vi "Main.vi"(11 "Module Admin":refnum<class "Delacor_lib_QMH_Module Admin.lvclass">) -> ()   [LabVIEW 2026, in "testCoordinator.lvlib"]
doc: "This template is based off of the Queued Message Handler design pattern and the Queued Message Handler project template that ships with LabVIEW.\n\nThe main difference is that the queue is private to this module and communication between modules is performed via Broadcast and Request events.\n\nRequest events are wrapped in public API methods and are handled in the Event Handling Loop (EHL) of this VI. Any module can register for Broadcast events sent by this module. The EHL generates messages based on user interface actions.\n\nThe Message Handling Loop (MHL) processes messages generated by the EHL, or by other messages. The messages are string values, so new messages can be added easily to the Message Cases case structure in the MHL. Each message cluster can also provide an optional value for Message Data, which is a variant that can be converted to whatever message-specific data is required.\n_____\nBased on DQMH Dev Tools: Project Template 7.1.2.1547."
uses:
  testCoordinator.lvlib
  <vilib>/Delacor/Delacor QMH/Libraries/Module Admin_class/Delacor_lib_QMH_Module Admin.lvclass
  Test Procedure.ctl
  modules/coordinator/src/Libraries/UserEventRecorder/TestEvent.ctl
  Module Data--cluster.ctl
  Do Something Argument--cluster.ctl
  <vilib>/Delacor/Delacor QMH/Libraries/Message Queue_class/Delacor_lib_QMH_Message Queue.lvclass/Delacor_lib_QMH_Message Queue.ctl
  Do Something Else Argument--cluster.ctl
  Do Something Else and Wait for Reply Argument--cluster.ctl
  Do Something Else and Wait (Reply Payload)--cluster.ctl
  Stop Argument--cluster.ctl
  <vilib>/Delacor/Delacor QMH/Libraries/Module Admin_class/Delacor_lib_QMH_Module Admin.lvclass/Delacor_lib_QMH_Module Admin.ctl
  Set Manual Tests Folder Location Argument--cluster.ctl
  Set Manual Tests Folder Location (Reply Payload)--cluster.ctl
  Load Test Procedure Argument--cluster.ctl
  Begin Test Execution Argument--cluster.ctl
  Process Test Procedure Metadata Argument--cluster.ctl
  Instruction Completed Argument--cluster.ctl
  Process First Instruction Argument--cluster.ctl
  Load Next Test Case Argument--cluster.ctl
  Execute Launcher Argument--cluster.ctl
  <vilib>/Utility/miscctls.llb/LVPointTypeDef.ctl
  modules/coordinator/src/Libraries/Launcher/Mode.ctl
  modules/ReplayMode.ctl
  modules/RecordMode.ctl
  <vilib>/Delacor/Delacor QMH/Libraries/Message Queue_class/Delacor_lib_QMH_Enqueue Message (Single).vi
  <vilib>/Delacor/Delacor QMH/Libraries/Module Admin_class/Delacor_lib_QMH_Get External Launch.vi
  modules/coordinator/src/Libraries/Core/global.vi
  <userlib>/_OpenG.lib/comparison/comparison.llb/String Changed__ogtk.vi
  <vilib>/Delacor/Delacor QMH/Libraries/Message Queue_class/Delacor_lib_QMH_Message Queue.lvclass
  modules/coordinator/src/Libraries/Launcher/Launcher.lvlib
  <userlib>/_OpenG.lib/comparison/comparison.llb/openg_comparison__ogtk.lvlib
panel:
  out "Array":T1[](array[typedef])
  in  "Exit":bool
  out "Scope":string
  out "TestProcedure":T2
  in  "Instruction Completed":bool
  out "Instruction":string
  out "Section":string
  out "Test Procedure":string
  out "error out":errorcluster
  out "X":dbl
  out "Status":string
  in  "Simulate MHL Error":bool
  in  "Simulate EHL Error":bool
  in  "Do Something Else <Replace Me>":bool
  in  "Do Something <Replace Me>":bool
  # "Open Visual Studio Code and run command \"LabVIEW Benchmark Actor: Capture LabVIEW Launch\" for the test to begin."
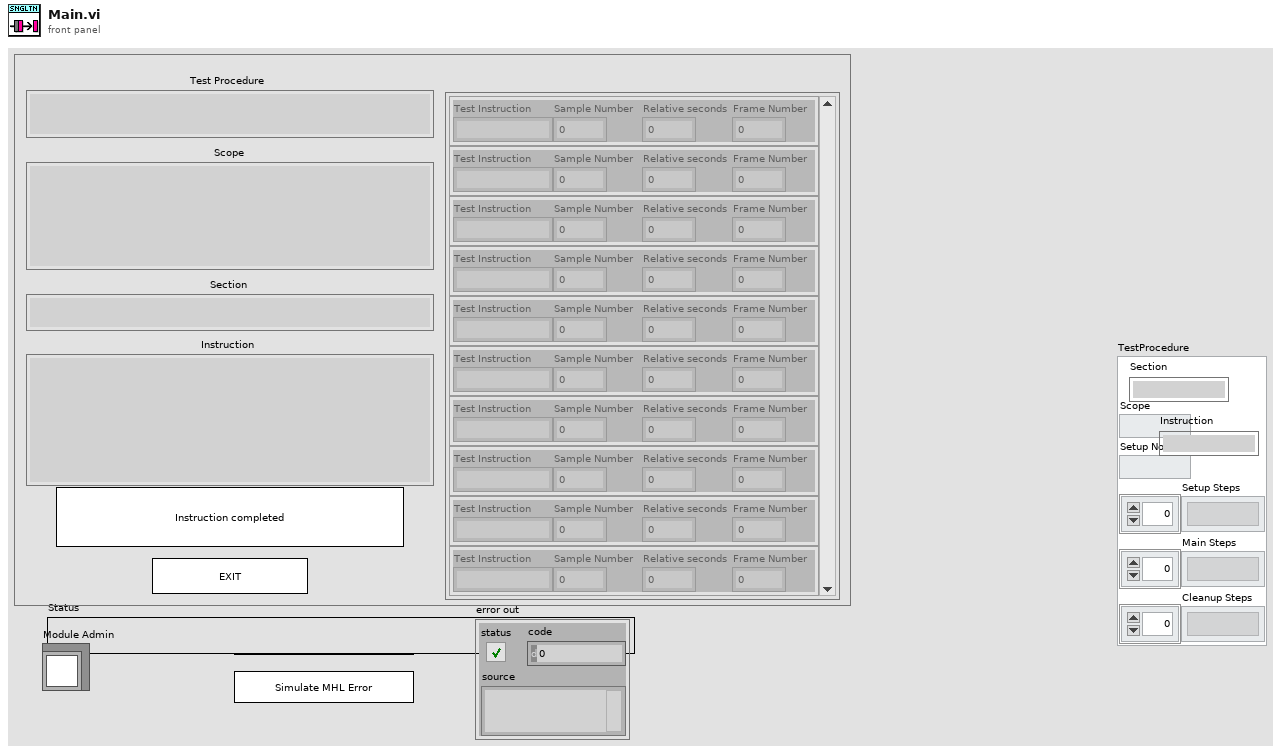
[diagram p1: front panel]
types:
  T1 = typedef "TestEvent.ctl" = cluster{"Test Instruction":string, "Sample Number":u32, "Relative seconds":dbl, "Frame Number":u32}
  T2 = typedef "Test Procedure.ctl" = cluster{"Scope":string, "Setup Note":string, "Setup Steps":string[], "Main Steps":string[], "Cleanup Steps":string[], "Section":string, "Instruction":string}
  T3 = typedef "testCoordinator.lvlib/Request Events--cluster.ctl" = cluster{"Stop Module":refnum<user-event>, "Do Something":refnum<user-event>, "Do Something Else":refnum<user-event>, "Do Something Else and Wait for Reply":refnum<user-event>, "Show Panel":refnum<user-event>, "Hide Panel":refnum<user-event>, "Get Module Execution Status":refnum<user-event>, "Show Diagram":refnum<user-event>, "Set Manual Tests Folder Location":refnum<user-event>, "Private.Load Test Procedure":refnum<user-event>, "Begin Test Execution":refnum<user-event>, "Private.Process Test Procedure Metadata":refnum<user-event>, "Private.Instruction Completed":refnum<user-event>, "Private.Process First Instruction":refnum<user-event>, "Private.Load Next Test Case":refnum<user-event>, "Private.Execute Launcher":refnum<user-event>}
  T4 = typedef "Launcher.lvlib/Broadcast Events--cluster.ctl" = cluster{"Module Did Init":refnum<user-event>, "Status Updated":refnum<user-event>, "Error Reported":refnum<user-event>, "Module Did Stop":refnum<user-event>, "Update Module Execution Status":refnum<user-event>, "Start Capture Detection Loop":refnum<user-event>, "Benchmark Started":refnum<user-event>, "Broadcast number of frames and run ID":refnum<user-event>}
  T5 = typedef "testCoordinator.lvlib/Module Data--cluster.ctl" = cluster{"Status":string, "Manual Tests Folder":path, "Available Tests":string[], "Test Procedure File Name":string, "TestCaseIndex":i32, "TestProcedure":T2}
  T6 = typedef "testCoordinator.lvlib/Do Something Argument--cluster.ctl" = cluster{"Do Something Msg":string}
  T7 = typedef "testCoordinator.lvlib/Do Something Else Argument--cluster.ctl" = cluster{"Do Something Else Msg":string, "X":dbl}
  T8 = typedef "testCoordinator.lvlib/Do Something Else and Wait for Reply Argument--cluster.ctl" = cluster{"Do Something Else Msg":string, "X":dbl, "Wait Notifier":refnum<notifier>, "wait for reply":bool}
  T9 = enum32{"invalid lock state", "Not Locked", "Locked (No Password)", "Password-protected"}
  T10 = typedef "testCoordinator.lvlib/Stop Argument--cluster.ctl" = cluster{"Origin":string, "Exit via Stop Module Req?":bool, "Wait for Module to stop?":bool}
  T11 = typedef "testCoordinator.lvlib/Set Manual Tests Folder Location Argument--cluster.ctl" = cluster{"Manual Tests Folder":path, "Wait Notifier":refnum<notifier>, "wait for reply":bool}
  T12 = typedef "testCoordinator.lvlib/Load Test Procedure Argument--cluster.ctl" = cluster{"Test Procedure File Name":string}
  T13 = typedef "testCoordinator.lvlib/Begin Test Execution Argument--cluster.ctl" = cluster{"Test Procedure":string}
  T14 = typedef "testCoordinator.lvlib/Process Test Procedure Metadata Argument--cluster.ctl" = cluster{"Boolean":bool}
  T15 = typedef "testCoordinator.lvlib/Instruction Completed Argument--cluster.ctl" = cluster{"Boolean":bool}
  T16 = typedef "testCoordinator.lvlib/Process First Instruction Argument--cluster.ctl" = cluster{"Boolean":bool}
  T17 = typedef "testCoordinator.lvlib/Load Next Test Case Argument--cluster.ctl" = cluster{"Boolean":bool}
  T18 = typedef "testCoordinator.lvlib/Execute Launcher Argument--cluster.ctl" = cluster{"Boolean":bool}
  T19 = typedef "LVPointTypeDef.ctl" = cluster{"Horizontal":i16, "Vertical":i16}
  T20 = enum32{"Invalid", "Standard", "Closed", "Hidden", "Minimized", "Maximized"}
  T21 = typedef "testCoordinator.lvlib/Do Something Else and Wait (Reply Payload)--cluster.ctl" = cluster{"Value":dbl, "error":errorcluster}
  T22 = typedef "testCoordinator.lvlib/Set Manual Tests Folder Location (Reply Payload)--cluster.ctl" = cluster{"Available Test Procedures":string[], "error":errorcluster}
  T23 = typedef "Mode.ctl" = cluster{"Replay":T24, "Record":T25}
  T24 = typedef "ReplayMode.ctl" = enum16{"None", "User Events"}
  T25 = typedef "RecordMode.ctl" = enum16{"None", "User Events", "Benchmarks", "User Events and Benchmarks"}
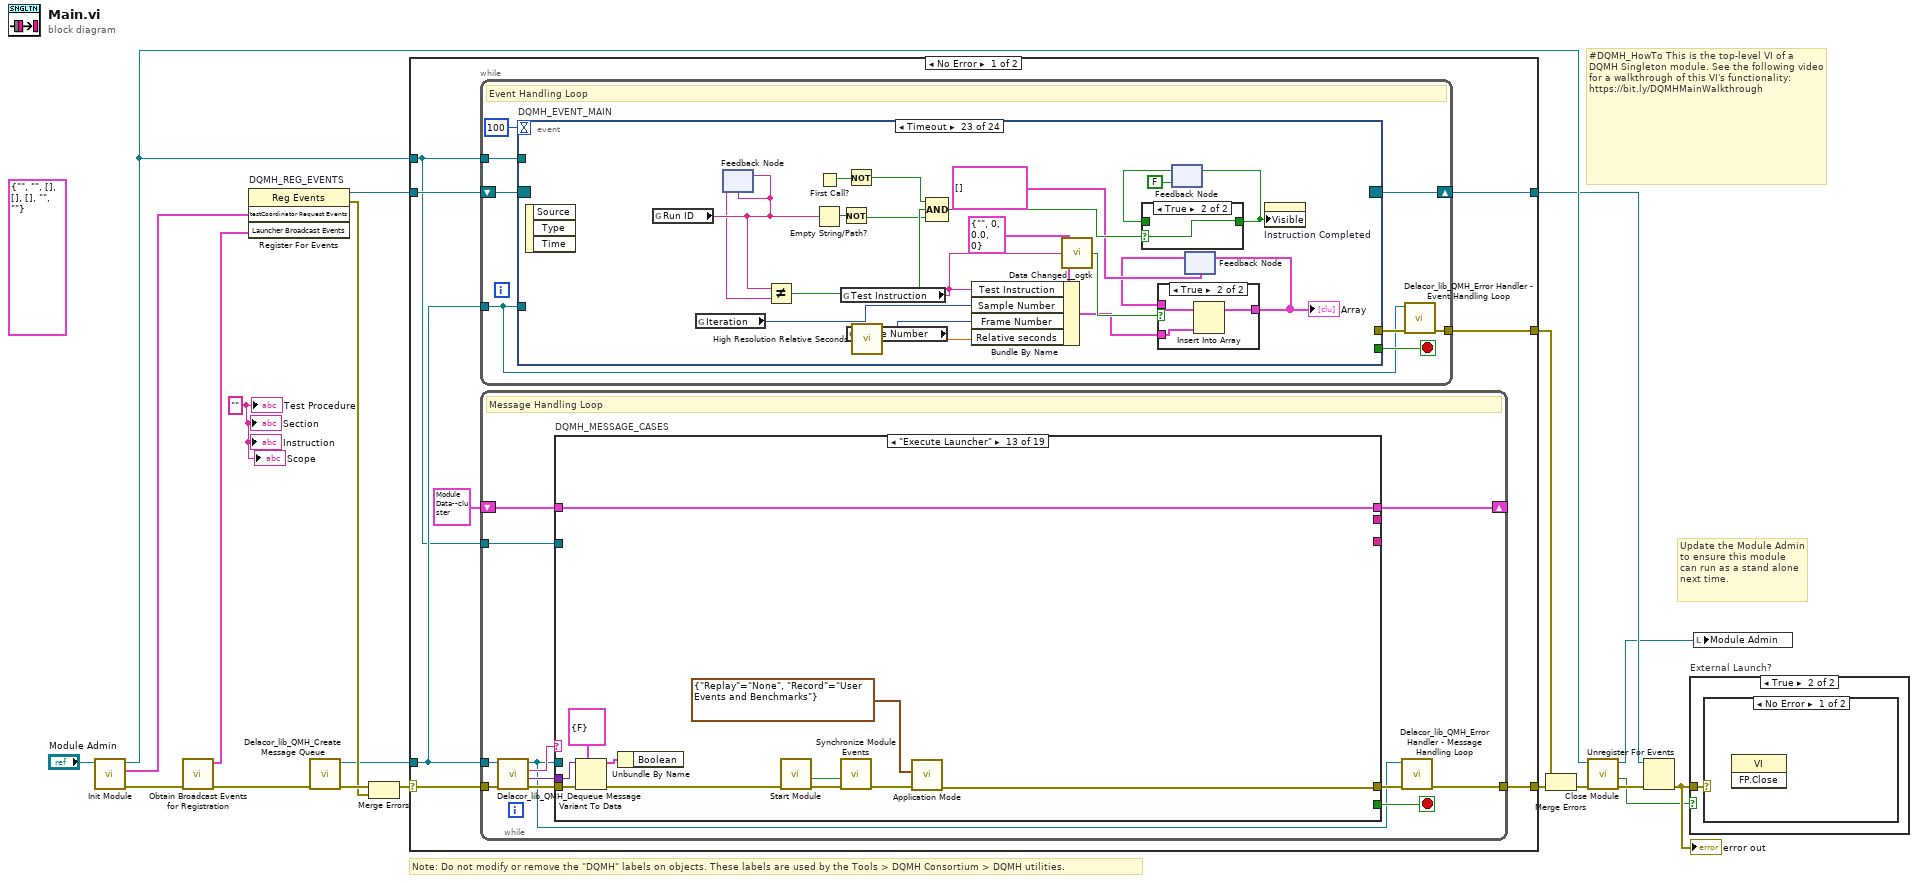
[diagram p0: block diagram]
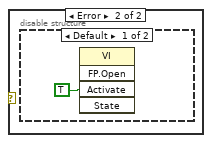
[diagram p3: hidden frame]
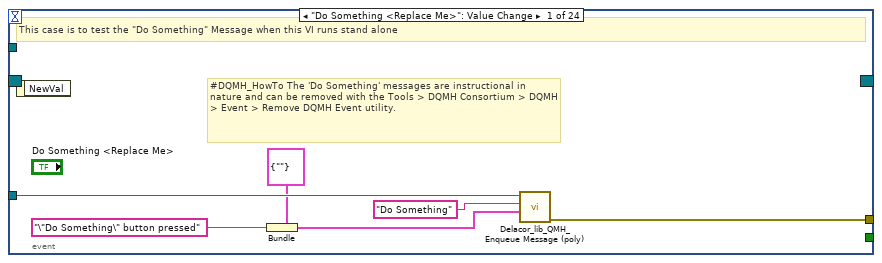
[diagram p5: hidden frame]
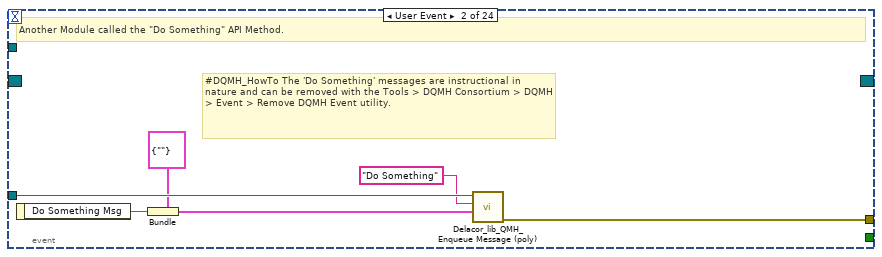
[diagram p6: hidden frame]
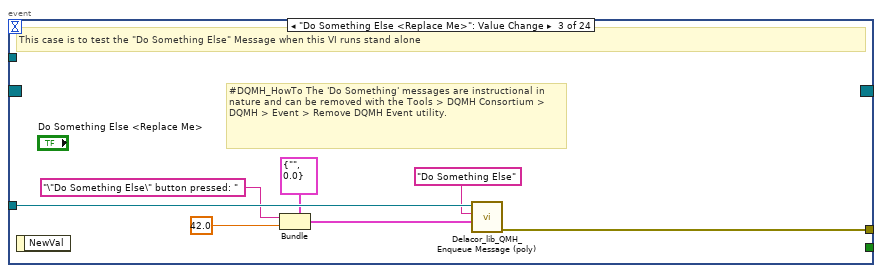
[diagram p7: hidden frame]
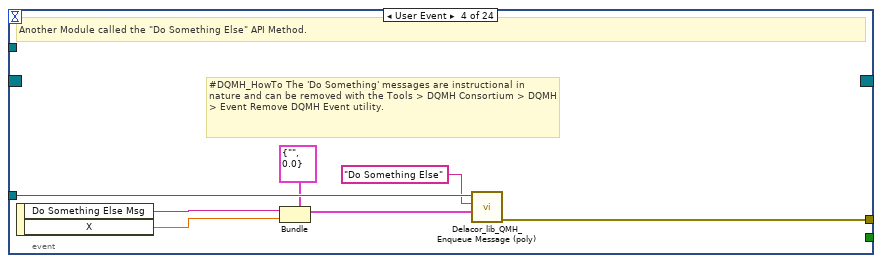
[diagram p8: hidden frame]
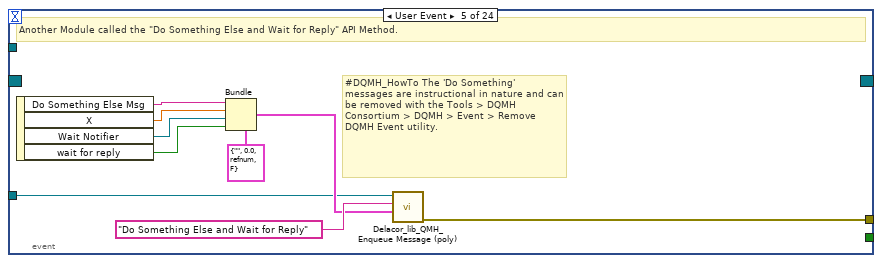
[diagram p9: hidden frame]
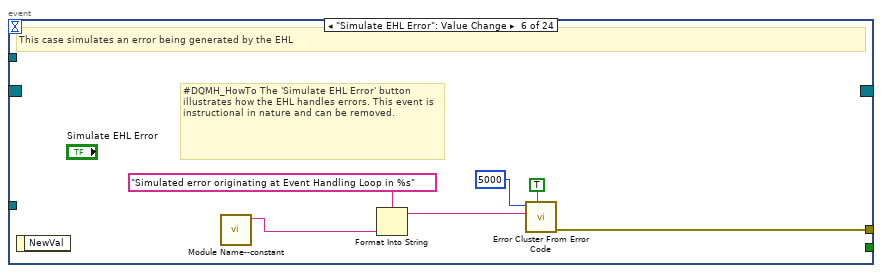
[diagram p10: hidden frame]
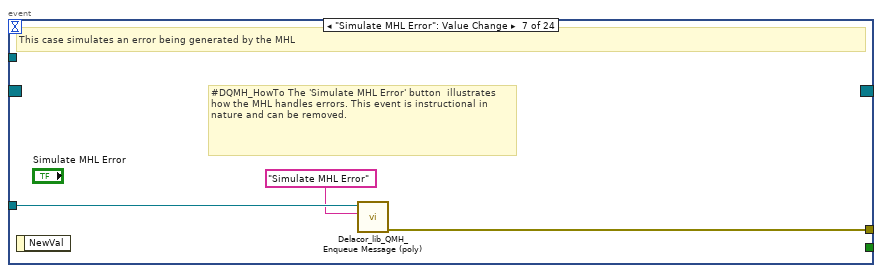
[diagram p11: hidden frame]
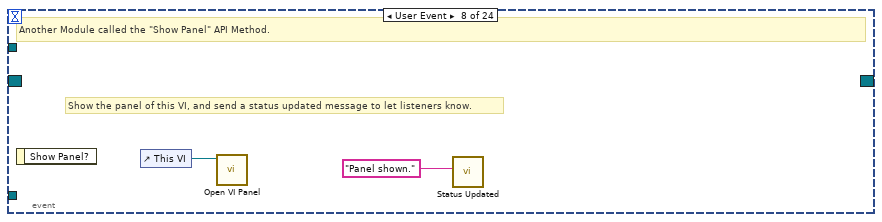
[diagram p12: hidden frame]
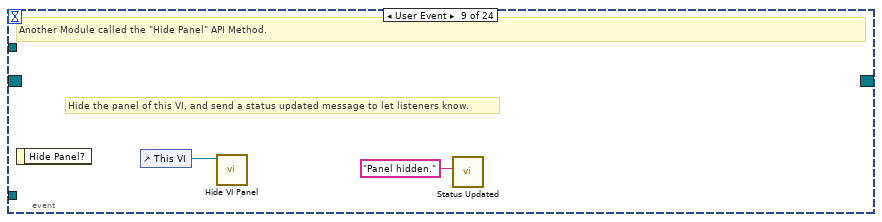
[diagram p13: hidden frame]
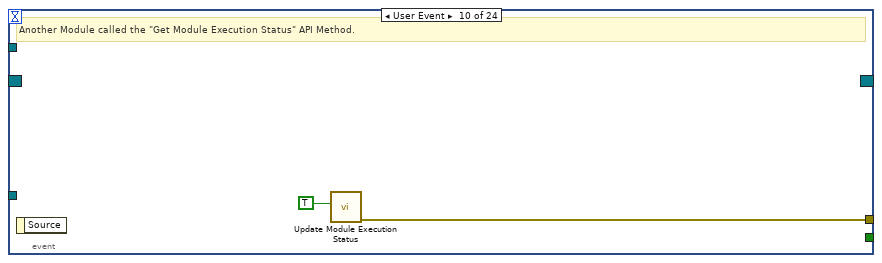
[diagram p14: hidden frame]
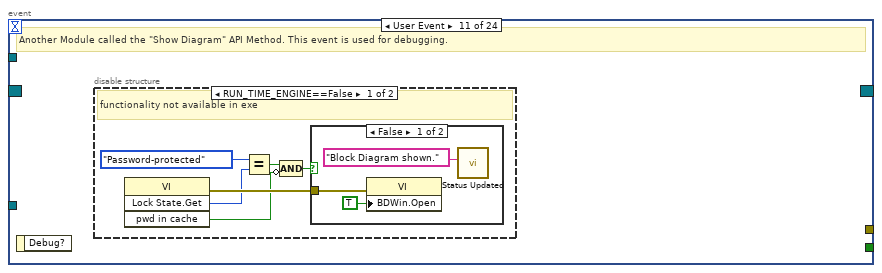
[diagram p15: hidden frame]
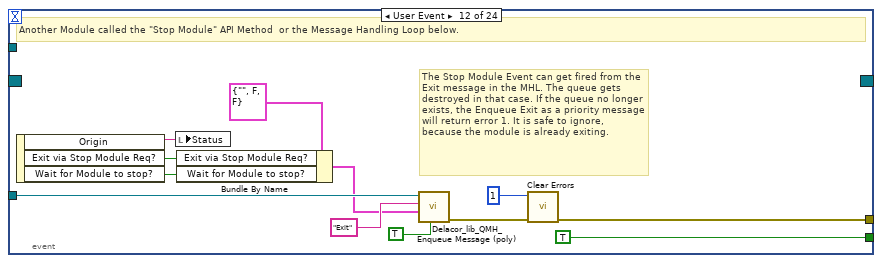
[diagram p18: hidden frame]
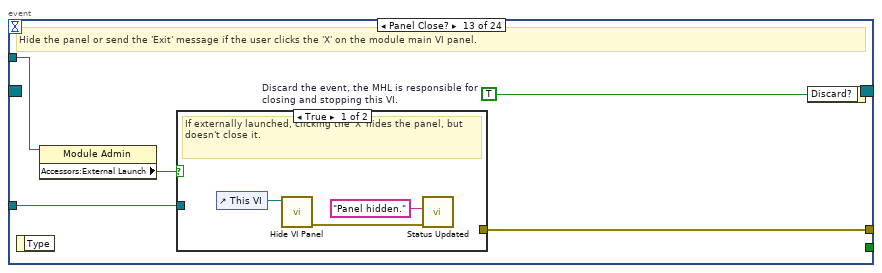
[diagram p19: hidden frame]
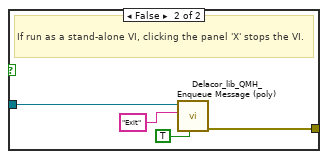
[diagram p20: hidden frame]
diagram:
  (unwired) T2 {"Scope"="", "Setup Note"="", "Setup Steps"=[], "Main Steps"=[], "Cleanup Steps"=[], "Section"="", "Instruction"=""} ("TestProcedure")
  w1 = "" ("Test Procedure")
  # "#DQMH_HowTo This is the top-level VI of a DQMH Singleton module. See the following video for a walkthrough of this VI's functionality: https://bit.ly/DQMHMainWalkthrough"
  # "Note: Do not modify or remove the \"DQMH\" labels on objects. These labels are used by the Tools > DQMH Consortium > DQMH utilities."
  # "Update the Module Admin to ensure this module can run as a stand alone next time."
  n1 = call "Init Module.vi"("Singleton Module Admin in"="Module Admin") -> ("error out"=w4:errorcluster, "testCoordinator Request Events"=w9:T3, "Singleton Module Admin out"=w12:refnum<class "Delacor_lib_QMH_Module Admin.lvclass">)  [unwired: 8 in]
  n2 = call "Obtain Broadcast Events for Registration.vi"("error in"=w4) -> ("error out"=w3:errorcluster, "Launcher Broadcast Events"=w2:T4)  [unwired: 8 in, 1 out]
  n3 = register-events "DQMH_REG_EVENTS"(w9, w2) -> (reference out=w10:refnum<event-registration>, error out=w13:errorcluster)  [unwired: 2 in]
  n4 = call <vilib>:"Delacor_lib_QMH_Create Message Queue.vi"("error in"=w3) -> ("error out"=w15:errorcluster, "Message Queue"=w8:refnum<class "Delacor_lib_QMH_Message Queue.lvclass">)  [unwired: 9 in]
  n5 = Merge Errors(w15, w13) -> (w14:errorcluster)
  n6 = case shown="No Error" w14 {
    selector: w14 -> [w26 w455]
    tunnel: [w28 w454] -> w20
    tunnel: [w25 w453] -> w11
    tunnel: w10 -> [w23 w453]
    tunnel: w8 -> [w22 w448]
    tunnel: [w27 _] -> w18
    tunnel: w12 -> [w21 w449]
    frame No Error {
      n7 = while {
        tunnel: w22 -> [w30]
        shift-right: [w33] -> w25
        shift-left: w23 -> [w34]
        tunnel: [w35] -> w27
        tunnel: w21 -> [w31]
        stop <- w32 stop-if-true
        # "Event Handling Loop"
        n8 = event "DQMH_EVENT_MAIN" shown="[22] Timeout" {
          selector: w34 -> [_ _ _ _ _ _ _ _ _ _ _ _ _ _ _ _ _ _ _ _ _ _ _ _]
          dyn-events: [_ _ _ _ _ _ _ _ _ _ _ _ _ _ _ _ _ _ _ _ _ _ _ _] -> w33
          timeout: 100 -> [_ _ _ _ _ _ _ _ _ _ _ _ _ _ _ _ _ _ _ _ _ _ _ _]
          tunnel: [_ _ _ _ _ _ _ _ _ _ _ TRUE ("Discard?") _ _ _ _ _ _ _ _ _ _ _ _] -> w32
          tunnel: w30 -> [w41 w47 w54 w61 w64 _ w79 _ _ _ _ w103 w110 w127 w133 w139 w145 w151 _ w158 w164 w170 _ _]
          tunnel: [w42 w48 w55 w62 w71 w77 w80 _ _ w86 _ w106 w112 w120 w128 w134 w140 w146 w152 w153 w159 w165 _ w198] -> w36
          tunnel: w31 -> [_ _ _ _ _ _ _ _ _ _ _ _ w109 _ _ _ _ _ _ _ _ _ _ _]
          event "Do Something <Replace Me>": Value Change {
            # "#DQMH_HowTo The 'Do Something' messages are instructional in nature and can be removed with the Tools > DQMH Consortium > DQMH > Event > Remove DQMH Event utility."
            # "This case is to test the \"Do Something\" Message when this VI runs stand alone"
            n9 = event-data() -> ()  [unwired: 1 in, 1 out]
            n10 = Bundle(cluster=T6 {"Do Something Msg"=""} ("Do Something Argument"), "Do Something Msg"="\"Do Something\" button pressed" ("\"Do Something\" button pressed")) -> (w37:T6)
            n11 = call-poly <vilib>:"Delacor_lib_QMH_Enqueue Message (poly).vi"("Message Data"=w37, "Message"="Do Something", "Message Queue in"=w41) -> ("error out"=w42:errorcluster)  [unwired: 7 in, 1 out]
          }
          event User Event {
            # "#DQMH_HowTo The 'Do Something' messages are instructional in nature and can be removed with the Tools > DQMH Consortium > DQMH > Event > Remove DQMH Event utility."
            # "Another Module called the \"Do Something\" API Method."
            n12 = event-data() -> ("Do Something Msg"=w44:string)  [unwired: 1 in]
            n13 = Bundle(cluster=T6 {"Do Something Msg"=""} ("Do Something Argument"), "Do Something Msg"=w44) -> (w43:T6)
            n14 = call-poly <vilib>:"Delacor_lib_QMH_Enqueue Message (poly).vi"("Message Data"=w43, "Message"="Do Something", "Message Queue in"=w47) -> ("error out"=w48:errorcluster)  [unwired: 7 in, 1 out]
          }
          event "Do Something Else <Replace Me>": Value Change {
            # "#DQMH_HowTo The 'Do Something' messages are instructional in nature and can be removed with the Tools > DQMH Consortium > DQMH > Event > Remove DQMH Event utility."
            # "This case is to test the \"Do Something Else\" Message when this VI runs stand alone"
            n15 = event-data() -> ()  [unwired: 1 in, 1 out]
            n16 = Bundle(cluster=T7 {"Do Something Else Msg"="", "X"=0.0} ("Do Something Else Argument"), "Do Something Else Msg"="\"Do Something Else\" button pressed: " ("\"Do Something Else\" button pressed"), "X"=42.0) -> (w51:T7)
            n17 = call-poly <vilib>:"Delacor_lib_QMH_Enqueue Message (poly).vi"("Message Data"=w51, "Message"="Do Something Else", "Message Queue in"=w54) -> ("error out"=w55:errorcluster)  [unwired: 7 in, 1 out]
          }
          event User Event {
            # "#DQMH_HowTo The 'Do Something' messages are instructional in nature and can be removed with the Tools > DQMH Consortium > DQMH > Event Remove DQMH Event utility."
            # "Another Module called the \"Do Something Else\" API Method."
            n18 = event-data() -> ("Do Something Else Msg"=w57:string, "X"=w56:dbl)  [unwired: 1 in]
            n19 = Bundle(cluster=T7 {"Do Something Else Msg"="", "X"=0.0} ("Do Something Else Argument"), "Do Something Else Msg"=w57, "X"=w56) -> (w58:T7)
            n20 = call-poly <vilib>:"Delacor_lib_QMH_Enqueue Message (poly).vi"("Message Data"=w58, "Message"="Do Something Else", "Message Queue in"=w61) -> ("error out"=w62:errorcluster)  [unwired: 7 in, 1 out]
          }
          event User Event {
            # "#DQMH_HowTo The 'Do Something' messages are instructional in nature and can be removed with the Tools > DQMH Consortium > DQMH > Event > Remove DQMH Event utility."
            # "Another Module called the \"Do Something Else and Wait for Reply\" API Method."
            n21 = event-data() -> ("Do Something Else Msg"=w67:string, "X"=w66:dbl, "Wait Notifier"=w65:refnum<notifier>, "wait for reply"=w63:bool)  [unwired: 1 in]
            n22 = Bundle(cluster=T8 {"Do Something Else Msg"="", "X"=0.0, "Wait Notifier"=refnum, "wait for reply"=FALSE} ("Do Something Else and Wait for Reply Argument"), "Do Something Else Msg"=w67, "X"=w66, "Wait Notifier"=w65, "wait for reply"=w63) -> (w68:T8)
            n23 = call-poly <vilib>:"Delacor_lib_QMH_Enqueue Message (poly).vi"("Message Data"=w68, "Message"="Do Something Else and Wait for Reply", "Message Queue in"=w64) -> ("error out"=w71:errorcluster)  [unwired: 7 in, 1 out]
          }
          event "Simulate EHL Error": Value Change {
            # "#DQMH_HowTo The 'Simulate EHL Error' button  illustrates how the EHL handles errors. This event is instructional in nature and can be removed."
            # "This case simulates an error being generated by the EHL"
            n24 = event-data() -> ()  [unwired: 1 in, 1 out]
            n25 = call "Module Name--constant.vi"() -> ("Module Name"=w74:string)  [unwired: 11 in]
            n26 = Format Into String(format string="Simulated error originating at Event Handling Loop in %s", w74) -> (resulting string=w75:string)  [unwired: 2 in, 1 out]
            n27 = call <vilib>:"Error Cluster From Error Code.vi"("show call chain? (False)"=TRUE, "error message (\"\")"=w75, "error code (0)"=5000) -> ("error out"=w77:errorcluster)  [unwired: 6 in]
          }
          event "Simulate MHL Error": Value Change {
            # "#DQMH_HowTo The 'Simulate MHL Error' button  illustrates how the MHL handles errors. This event is instructional in nature and can be removed."
            # "This case simulates an error being generated by the MHL"
            n28 = event-data() -> ()  [unwired: 1 in, 1 out]
            n29 = call-poly <vilib>:"Delacor_lib_QMH_Enqueue Message (poly).vi"("Message"="Simulate MHL Error", "Message Queue in"=w79) -> ("error out"=w80:errorcluster)  [unwired: 8 in, 1 out]
          }
          event User Event {
            # "Show the panel of this VI, and send a status updated message to let listeners know."
            # "Another Module called the \"Show Panel\" API Method."
            n30 = event-data() -> ()  [unwired: 1 in, 1 out]
            n31 = control-ref of="This VI"() -> (w82:refnum<vi>)
            n32 = call "Open VI Panel.vi"("VI"=w82) -> ()  [unwired: 10 in, 1 out]
            n33 = call "Status Updated.vi"("Status"="Panel shown." ("format string")) -> ()  [unwired: 10 in, 1 out]
          }
          event User Event {
            # "Hide the panel of this VI, and send a status updated message to let listeners know."
            # "Another Module called the \"Hide Panel\" API Method."
            n34 = event-data() -> ()  [unwired: 1 in, 1 out]
            n35 = control-ref of="This VI"() -> (w84:refnum<vi>)
            n36 = call "Hide VI Panel.vi"("VI"=w84) -> ()  [unwired: 10 in, 1 out]
            n37 = call "Status Updated.vi"("Status"="Panel hidden." ("format string")) -> ()  [unwired: 10 in, 1 out]
          }
          event User Event {
            # "Another Module called the \"Get Module Execution Status\" API Method."
            n38 = event-data() -> ()  [unwired: 1 in, 1 out]
            n39 = call "Update Module Execution Status.vi"("Running?"=TRUE) -> ("error out"=w86:errorcluster)  [unwired: 10 in]
          }
          event User Event {
            # "Another Module called the \"Show Diagram\" API Method. This event is used for debugging."
            n40 = event-data() -> ()  [unwired: 1 in, 1 out]
            n41 = disable-structure shown="RUN_TIME_ENGINE==False" {
              frame condition #0 (active) {
                # "functionality not available in exe"
                n42 = invoke on="Invoke Node" class="VI" method="Lock State.Get"() -> (error out=w92:errorcluster, "Get Lock State"=w91:T9, "pwd in cache"=w88:bool)  [unwired: 4 in, 1 out]
                n43 = Equal?(x=T9."Password-protected", y=w91) -> (x = y?=w89:bool)
                n44 = Compound Arithmetic op=AND(w89, invert w88) -> (w87:bool)
                n45 = case shown="False" w87 {
                  tunnel: w92 -> [w95 _]
                  frame False {
                    n46 = property on="Property Node" class="VI"(error in=w95, "BDWin.Open"=TRUE ("Block Diagram Window:Open")) -> ()  [unwired: 1 in, 2 out]
                    n47 = call "Status Updated.vi"("Status"="Block Diagram shown." ("format string")) -> ()  [unwired: 10 in, 1 out]
                  }
                  frame True {
                    # "Password-protected VI, and the password is not in the cache. Do not show the diagram."
                  }
                }
              }
              frame condition #1 {
              }
            }
          }
          event User Event {
            # "The Stop Module Event can get fired from the Exit message in the MHL. The queue gets destroyed in that case. If the queue no longer exists, the Enqueue Exit as a priority message will return error 1. It is safe to ignore, because the module is already exiting."
            # "Another Module called the \"Stop Module\" API Method  or the Message Handling Loop below."
            n48 = event-data() -> ("Origin"=w102:string, "Exit via Stop Module Req?"=w98:bool, "Wait for Module to stop?"=w97:bool)  [unwired: 1 in]
            n49 = local write "Status"(w102) -> ()
            n50 = Bundle By Name(cluster=T10 {"Origin"="", "Exit via Stop Module Req?"=FALSE, "Wait for Module to stop?"=FALSE} ("Stop Argument"), "Exit via Stop Module Req?"=w98, "Wait for Module to stop?"=w97) -> (w96:T10)
            n51 = call-poly <vilib>:"Delacor_lib_QMH_Enqueue Message (poly).vi"("Priority Message? (F)"=TRUE, "Message Data"=w96, "Message"="Exit", "Message Queue in"=w103) -> ("error out"=w107:errorcluster)  [unwired: 6 in, 1 out]
            n52 = call <vilib>:"Clear Errors.vi"("error in (no error)"=w107, "specific error code to clear (0: all)"=1) -> ("error out"=w106:errorcluster)  [unwired: 4 in, 1 out]
          }
          event Panel Close? {
            w111 = TRUE  # Discard the event, the MHL is responsible for closing and stopping this VI.
            # "Hide the panel or send the 'Exit' message if the user clicks the 'X' on the module main VI panel."
            n53 = event-data() -> ()  [unwired: 1 in, 1 out]
            n54 = property on="Property Node" class="Module Admin"(reference=w109) -> ("Accessors:External Launch"=w108:bool)  [unwired: 1 in, 2 out]
            n55 = case shown="True" w108 {
              tunnel: w110 -> [_ w118]
              tunnel: [_ w119] -> w112
              frame True {
                # "If externally launched, clicking the 'X' hides the panel, but doesn't close it."
                n56 = control-ref of="This VI"() -> (w115:refnum<vi>)
                n57 = call "Hide VI Panel.vi"("VI"=w115) -> ("error out"=w113:errorcluster)  [unwired: 10 in]
                n58 = call "Status Updated.vi"("error in"=w113, "Status"="Panel hidden." ("format string")) -> ()  [unwired: 9 in, 1 out]
              }
              frame False {
                # "If run as a stand-alone VI, clicking the panel 'X' stops the VI."
                n59 = call-poly <vilib>:"Delacor_lib_QMH_Enqueue Message (poly).vi"("Priority Message? (F)"=TRUE, "Message"="Exit", "Message Queue in"=w118) -> ("error out"=w119:errorcluster)  [unwired: 7 in, 1 out]
              }
            }
            n60 = event-data ("Event Filter Node")("Discard?"=w111) -> ()  [unwired: 1 in, 1 out]
          }
          event User Event {
            # "Another Module called the \"Set Manual Tests Folder Location\" API Method."
            n61 = event-data() -> ("Manual Tests Folder"=w123:path, "Wait Notifier"=w122:refnum<notifier>, "wait for reply"=w121:bool)  [unwired: 1 in]
            n62 = Bundle(cluster=T11 {"Manual Tests Folder"=path "", "Wait Notifier"=refnum, "wait for reply"=FALSE} ("Set Manual Tests Folder Location Argument"), "Manual Tests Folder"=w123, "Wait Notifier"=w122, "wait for reply"=w121) -> (w124:T11)
            n63 = call-poly <vilib>:"Delacor_lib_QMH_Enqueue Message (poly).vi"("Message Data"=w124, "Message"="Set Manual Tests Folder Location", "Message Queue in"=w127) -> ("error out"=w120:errorcluster)  [unwired: 7 in, 1 out]
          }
          event User Event {
            # "This module called the \"Private.Load Test Procedure\" private request."
            n64 = event-data() -> ("Test Procedure File Name"=w129:string)  [unwired: 1 in]
            n65 = Bundle(cluster=T12 {"Test Procedure File Name"=""} ("Load Test Procedure Argument"), "Test Procedure File Name"=w129) -> (w130:T12)
            n66 = call-poly <vilib>:"Delacor_lib_QMH_Enqueue Message (poly).vi"("Message Data"=w130, "Message"="Load Test Procedure", "Message Queue in"=w133) -> ("error out"=w128:errorcluster)  [unwired: 7 in, 1 out]
          }
          event User Event {
            # "Another Module called the \"Begin Test Execution\" API Method."
            n67 = event-data() -> ("Test Procedure"=w135:string)  [unwired: 1 in]
            n68 = Bundle(cluster=T13 {"Test Procedure"=""} ("Begin Test Execution Argument"), "Test Procedure"=w135) -> (w136:T13)
            n69 = call-poly <vilib>:"Delacor_lib_QMH_Enqueue Message (poly).vi"("Message Data"=w136, "Message"="Begin Test Execution", "Message Queue in"=w139) -> ("error out"=w134:errorcluster)  [unwired: 7 in, 1 out]
          }
          event User Event {
            # "This module called the \"Private.Process Test Procedure Metadata\" private request."
            n70 = event-data() -> ("Boolean"=w141:bool)  [unwired: 1 in]
            n71 = Bundle(cluster=T14 {"Boolean"=FALSE} ("Process Test Procedure Metadata Argument"), "Boolean"=w141) -> (w142:T14)
            n72 = call-poly <vilib>:"Delacor_lib_QMH_Enqueue Message (poly).vi"("Message Data"=w142, "Message"="Process Test Procedure Metadata", "Message Queue in"=w145) -> ("error out"=w140:errorcluster)  [unwired: 7 in, 1 out]
          }
          event User Event {
            # "This module called the \"Private.Instruction Completed\" private request."
            n73 = event-data() -> ("Boolean"=w147:bool)  [unwired: 1 in]
            n74 = Bundle(cluster=T15 {"Boolean"=FALSE} ("Instruction Completed Argument"), "Boolean"=w147) -> (w148:T15)
            n75 = call-poly <vilib>:"Delacor_lib_QMH_Enqueue Message (poly).vi"("Message Data"=w148, "Message"="Instruction Completed", "Message Queue in"=w151) -> ("error out"=w146:errorcluster)  [unwired: 7 in, 1 out]
          }
          event "Instruction Completed": Value Change {
            n76 = event-data() -> ()  [unwired: 1 in, 1 out]
            n77 = call "Instruction Completed.vi"() -> ("error out"=w152:errorcluster)  [unwired: 11 in]
          }
          event User Event {
            # "This module called the \"Private.Process First Instruction\" private request."
            n78 = event-data() -> ("Boolean"=w154:bool)  [unwired: 1 in]
            n79 = Bundle(cluster=T16 {"Boolean"=FALSE} ("Process First Instruction Argument"), "Boolean"=w154) -> (w155:T16)
            n80 = call-poly <vilib>:"Delacor_lib_QMH_Enqueue Message (poly).vi"("Message Data"=w155, "Message"="Process First Instruction", "Message Queue in"=w158) -> ("error out"=w153:errorcluster)  [unwired: 7 in, 1 out]
          }
          event User Event {
            # "This module called the \"Private.Load Next Test Case\" private request."
            n81 = event-data() -> ("Boolean"=w160:bool)  [unwired: 1 in]
            n82 = Bundle(cluster=T17 {"Boolean"=FALSE} ("Load Next Test Case Argument"), "Boolean"=w160) -> (w161:T17)
            n83 = call-poly <vilib>:"Delacor_lib_QMH_Enqueue Message (poly).vi"("Message Data"=w161, "Message"="Load Next Test Case", "Message Queue in"=w164) -> ("error out"=w159:errorcluster)  [unwired: 7 in, 1 out]
          }
          event User Event {
            # "This module called the \"Private.Execute Launcher\" private request."
            n84 = event-data() -> ("Boolean"=w166:bool)  [unwired: 1 in]
            n85 = Bundle(cluster=T18 {"Boolean"=FALSE} ("Execute Launcher Argument"), "Boolean"=w166) -> (w167:T18)
            n86 = call-poly <vilib>:"Delacor_lib_QMH_Enqueue Message (poly).vi"("Message Data"=w167, "Message"="Execute Launcher", "Message Queue in"=w170) -> ("error out"=w165:errorcluster)  [unwired: 7 in, 1 out]
          }
          event Timeout {
            n87 = event-data() -> ()  [unwired: 1 in, 3 out]
            n88 = global read "global.vi" "Run ID"() -> (w188:string)
            n89 = global read "global.vi" "Iteration"() -> (w179:u64)
            n90 = feedback-in #1(w188) -> ()
            n91 = feedback #1(w188) -> (w187:string)
            n92 = Not Equal?(x=w188, y=w187) -> (x != y?=w186:bool)
            n93 = Empty String/Path?(string/path=w188) -> (empty?=w191:bool)
            n94 = First Call?() -> (First Call?: T/F=w190:bool)
            n95 = Not(x=w191) -> (.not. x?=w185:bool)
            n96 = global read "global.vi" "Test Instruction"() -> (w176:string)
            n97 = Not(x=w190) -> (.not. x?=w189:bool)
            n98 = global read "global.vi" "Frame Number"() -> (w178:u32)
            n99 = call <vilib>:"High Resolution Relative Seconds.vi"() -> ("relative seconds"=w177:dbl)
            n100 = Compound Arithmetic op=AND(w189, w186, w185) -> (w184:bool)
            n101 = Bundle By Name(cluster=T1 {"Test Instruction"="", "Sample Number"=0, "Relative seconds"=0.0, "Frame Number"=0} ("TestEvent"), "Test Instruction"=w176, "Sample Number"=w179, "Frame Number"=w178, "Relative seconds"=w177) -> (w174:T1)
            n102 = call-poly <userlib>:"Data Changed__ogtk.vi"("String"=w176) -> ("Changed"=w175:bool)
            n103 = feedback #2(FALSE) -> (w183:bool)
            n104 = case shown="True" w184 {
              selector: w184 -> [_ w197]
              tunnel: w183 -> [w196 _]
              tunnel: [w196 w197] -> w181
              frame False {
              }
              frame True {
              }
            }
            n105 = feedback-in #2(w181) -> ()
            n106 = feedback #3(T1[] [] ("Array")) -> (w172:T1[])
            n107 = case shown="True" w175 {
              tunnel: w174 -> [_ w194]
              tunnel: w172 -> [w192 w195]
              tunnel: [w192 w193] -> w171
              frame False {
              }
              frame True {
                n108 = Insert Into Array(array=w195, new element=w194) -> (w193:T1[])  [unwired: 1 in]
              }
            }
            "Array" <- w171
            n109 = feedback-in #3(w171) -> ()
            n110 = property on="Instruction Completed" class="Bool"("Visible"=w181) -> ()  [unwired: 2 in, 2 out]
          }
          event "Exit": Value Change {
            n111 = event-data() -> ()  [unwired: 1 in, 6 out]
            n112 = call "Stop Module.vi"() -> ("error out"=w198:errorcluster)  [unwired: 11 in]
          }
        }
        n113 = call-dynamic "Delacor_lib_QMH_Error Handler - Event Handling Loop.vi"("error in"=w36, "Message Queue in"=w30) -> ("dup error in"=w35:errorcluster)  [unwired: 8 in, 1 out]
      }
      n114 = while {
        tunnel: w22 -> [w199]
        shift-right: [w207] -> _
        shift-left: T5 {"Status"="", "Manual Tests Folder"=path "", "Available Tests"=[], "Test Procedure File Name"="", "TestCaseIndex"=0, "TestProcedure"={"Scope"="", "Setup Note"="", "Setup Steps"=[], "Main Steps"=[], "Cleanup Steps"=[], "Section"="", "Instruction"=""}} ("Data Cluster") -> [w208]
        tunnel: w26 -> [w210]
        tunnel: [w202] -> w28
        tunnel: w21 -> [w203]
        stop <- w206 stop-if-true
        # "Message Handling Loop"
        n115 = call-dynamic "Delacor_lib_QMH_Dequeue Message.vi"("error in"=w210, "Message Queue in"=w199) -> ("error out"=w209:errorcluster, "Message Data"=w204:variant, "Message"=w205:string, "Message Queue out"=w200:refnum<class "Delacor_lib_QMH_Message Queue.lvclass">)  [unwired: 6 in]
        n116 = case "DQMH_MESSAGE_CASES" shown="\"Execute Launcher\"" w205 {
          selector: w205 -> [_ _ _ _ _ _ _ _ _ _ _ _ _ _ _ _ _ _ w443]
          tunnel: w200 -> [_ _ _ _ _ _ _ _ _ _ _ _ _ _ _ _ w405 w431 _]
          tunnel: w209 -> [w228 w232 w240 w249 w268 w300 w310 w320 w331 w339 w360 w372 w387 w390 w392 w401 w412 w437 w446]
          tunnel: [w226 w232 w238 w248 w267 w291 w309 w313 w330 w332 w359 w371 w377 w389 w392 w400 w408 w432 w447] -> w201
          tunnel: w208 -> [w217 w231 w237 w247 w264 w290 w305 w316 w324 w335 w349 w365 w386 w388 w391 w398 w407 w430 w444]
          tunnel: [w216 w231 w237 w247 w264 w289 w304 w315 w323 w334 w348 w365 w386 w388 w391 w398 w407 w430 w444] -> w207
          tunnel: [_ _ _ _ _ _ _ _ _ _ _ _ _ _ _ _ _ w429 _] -> w206
          tunnel: w204 -> [_ _ w236 w244 w261 w298 w308 w319 w329 w338 w358 w370 w385 _ _ _ w406 w428 _]
          tunnel: w203 -> [w218 _ _ _ _ _ _ _ _ _ _ _ _ _ _ _ w404 w423 _]
          tunnel: [_ _ _ _ _ _ _ _ _ _ _ w362 _ _ _ _ _ _ _] -> _
          tunnel: [_ _ _ _ _ _ _ _ _ _ w345 w363 _ _ _ _ _ _ _] -> _
          frame "Initialize" {
            (unwired) string[][] [] ("Item Names")
            w212 = "Initial Message" ("Initial Message")
            # "#DQMH_CodeNeeded - Initialize the appearance of the front panel."
            # "#DQMH_CodeNeeded - Initialize your state data here."
            # "Initialize - Any operation that needs to be done before the module can receive messages. Synchronize Caller Events.vi will inform Start Module.vi that the module has launched and is ready to receive messages. Module Did Init.vi will broadcast that the module initialized."
            n117 = call "Synchronize Caller Events.vi"("error in"=w228, "Singleton Module Admin in"=w218) -> ("error out"=w227:errorcluster, "Singleton Module Admin out"=w213:refnum<class "Delacor_lib_QMH_Module Admin.lvclass">)  [unwired: 8 in]
            n118 = property on="Property Node" class="Module Admin"(reference=w213) -> ("Accessors:External Launch"=w222:bool)  [unwired: 1 in, 2 out]
            n119 = Select(t=T20."Hidden" ("State"), s=w222, f=T20."Standard" ("State")) -> (s? t:f=w219:T20)
            n120 = call "Module Name--constant.vi"() -> ("Module Name"=w225:string)  [unwired: 11 in]
            n121 = property on="Property Node" class="VI"("Front Panel.Title"=w225) -> (reference out=w224:refnum<vi>, error out=w230:errorcluster)  [unwired: 2 in]
            n122 = invoke on="Invoke Node" class="VI" method="FP.Open"(reference=w224, error in=w230, "State"=w219) -> (reference out=w223:refnum<vi>, error out=w229:errorcluster)  [unwired: 2 in, 3 out]
            n123 = Bundle By Name(cluster=w217, "Status"=w212) -> (w216:T5)
            n124 = invoke on="Invoke Node" class="VI" method="FP.Center"(reference=w223, error in=w229) -> ()  [unwired: 1 in, 3 out]
            n125 = property on="Pane" class="Pane"("Origin"=T19 {"Horizontal"=0, "Vertical"=0}) -> ()  [unwired: 2 in, 2 out]
            n126 = call "Module Name--constant.vi"() -> ("Module Name"=w214:string)  [unwired: 11 in]
            n127 = call "Module Did Init.vi"("error in"=w227, "Initialized?"=TRUE, "Origin"=w214) -> ("error out"=w226:errorcluster)  [unwired: 8 in]
            "Status" <- w212
          }
          frame "---Module Specific---" {
            # "Separator -- The following cases handle messages specific to this Module."
          }
          frame "Do Something" {
            # "#DQMH_HowTo The 'Do Something' messages are instructional in nature and can be removed with the Tools > DQMH Consortium > DQMH > Event > Remove DQMH Event utility."
            # "Do Something - Replace this message with functionality for your own application. Note that this message also fires the \"Did Something\" broadcast event."
            n128 = Variant To Data(error in=w240, type=T6 {"Do Something Msg"=""} ("Do Something Argument"), Variant=w236) -> (data=w235:T6, error out=w239:errorcluster)
            n129 = Unbundle By Name(w235) -> ("Do Something Msg"=w233:string)
            n130 = call "Did Something.vi"("error in"=w239, "Did Something Msg"=w233) -> ("error out"=w238:errorcluster)  [unwired: 9 in]
            n131 = local write "Status"(w233) -> ()
            n132 = call "Status Updated.vi"("Status"=w233) -> ()  [unwired: 10 in, 1 out]
          }
          frame "Do Something Else" {
            # "#DQMH_HowTo The 'Do Something' messages are instructional in nature and can be removed with the Tools > DQMH Consortium > DQMH > Event > Remove DQMH Event utility."
            # "Do Something Else - Replace this message with functionality for your own application."
            n133 = Variant To Data(error in=w249, type=T7 {"Do Something Else Msg"="", "X"=0.0} ("Do Something Else Argument"), Variant=w244) -> (data=w245:T7, error out=w248:errorcluster)
            n134 = Unbundle By Name(w245) -> ("Do Something Else Msg"=w243:string, "X"=w242:dbl)
            "X" <- w242
            n135 = Format Into String(initial string=w243, w242) -> (resulting string=w241:string)  [unwired: 2 in, 1 out]
            n136 = local write "Status"(w241) -> ()
            n137 = call "Status Updated.vi"("Status"=w241) -> ()  [unwired: 10 in, 1 out]
          }
          frame "Do Something Else and Wait for Reply" {
            w256 = "X(%.2f)+Offset(%.2f)=%.2f"  # status message format string
            # "#DQMH_HowTo The 'Do Something' messages are instructional in nature and can be removed."
            # "Send back X with a random offset"
            # "Do Something Else and Wait for Reply - Replace this message with functionality for your own application. Note that this message must fire a notifier to let callers know it has finished execution, and it returns an error if the 'Value' is negative."
            n138 = Variant To Data(error in=w268, type=T8 {"Do Something Else Msg"="", "X"=0.0, "Wait Notifier"=refnum, "wait for reply"=FALSE} ("Do Something Else and Wait for Reply Argument"), Variant=w261) -> (data=w262:T8, error out=w266:errorcluster)
            n139 = Unbundle By Name(w262) -> ("Wait Notifier"=w250:refnum<notifier>, "Do Something Else Msg"=w260:string, "X"=w257:dbl, "wait for reply"=w253:bool)
            n140 = Random Number (0-1)() -> (number: 0 to 1=w258:dbl)
            n141 = Add(x=w258, y=w257) -> (x+y=w252:dbl)
            n142 = Less Than 0?(x=w252) -> (x < 0?=w255:bool)
            n143 = local write "X"(w257) -> ()
            n144 = case shown="True" w255 {
              tunnel: [_ w278] -> w265
              frame False {
              }
              frame True {
                n145 = call <vilib>:"Error Cluster From Error Code.vi"("show call chain? (False)"=TRUE, "error message (\"\")"="The 'Something Else and Wait for Reply' message generated a negative number, which is considered an error condition.", "error code (0)"=5000) -> ("error out"=w278:errorcluster)  [unwired: 6 in]
              }
            }
            n146 = Format Into String(format string=w256, initial string=w260, w257, w258, w252) -> (resulting string=w254:string)  [unwired: 1 in, 1 out]
            n147 = Bundle By Name(cluster=T21 {"Value"=0.0, "error"={"status"=FALSE, "code"=0, "source"=""}} ("notification"), "error"=w265, "Value"=w252) -> (w251:T21)
            n148 = local write "Status"(w254) -> ()
            n149 = call "Status Updated.vi"("Status"=w254) -> ()  [unwired: 10 in, 1 out]
            n150 = case shown="True" w253 {
              tunnel: w251 -> [_ w271]
              tunnel: w250 -> [_ w270]
              frame False {
              }
              frame True {
                # "Simulate an operation that requires a wait."
                n151 = flat-sequence {
                  tunnel: w271 -> [w274]
                  tunnel: w270 -> [w273]
                  tunnel: w269 -> [_]
                  frame #0 {
                    n152 = Send Notification(notification=w274, notifier=w273) -> ()  [unwired: 1 in, 2 out]
                  }
                }
                n153 = Wait (ms)(milliseconds to wait=u32 1000) -> (millisecond timer value=w269:u32)
              }
            }
            n154 = Merge Errors(w266, w265) -> (w267:errorcluster)
          }
          frame "Set Manual Tests Folder Location" {
            # "Populates multicolumn listbox with compatible .md files"
            n155 = Variant To Data(error in=w300, type=T11 {"Manual Tests Folder"=path "", "Wait Notifier"=refnum, "wait for reply"=FALSE} ("Set Manual Tests Folder Location Argument"), Variant=w298) -> (data=w296:T11, error out=w299:errorcluster)
            n156 = Unbundle By Name(w296) -> ("Manual Tests Folder"=w287:path, "Wait Notifier"=w295:refnum<notifier>, "wait for reply"=w294:bool)
            n157 = List Folder(path=w287, pattern="*.md") -> (path out=w286:path, filenames=w280:string[], error out=w282:errorcluster)  [unwired: 2 in, 1 out]
            n158 = Build Array(w280) -> (w281:string[][])
            n159 = Array Size(array=w280) -> (size(s)=w285:i32)
            n160 = Transpose 2D Array(2D array=w281) -> (transposed array=w279:string[][])
            n161 = Format Into String(format string="Loaded %d Tests", w285) -> (resulting string=w283:string)  [unwired: 2 in, 1 out]
            n162 = Bundle By Name(cluster=T22 {"Available Test Procedures"=[], "error"={"status"=FALSE, "code"=0, "source"=""}} ("Set Manual Tests Folder Location (Reply Payload)"), "Available Test Procedures"=w280, "error"=w282) -> (w293:T22)
            n163 = Merge Errors(w299, w282) -> (w291:errorcluster)
            n164 = call "Broadcast Available Tests.vi"("Available Tests"=w279) -> ()  [unwired: 10 in, 1 out]
            n165 = Bundle By Name(cluster=w290, "Available Tests"=w280, "Manual Tests Folder"=w286, "Status"=w283) -> (w289:T5)
            n166 = case "DQMH_FIRE_NOTIFIER" shown="True" w294 {
              tunnel: w295 -> [_ w302]
              tunnel: w293 -> [_ w301]
              frame False {
              }
              frame True {
                n167 = Send Notification(notification=w301, notifier=w302) -> ()  [unwired: 1 in, 2 out]
              }
            }
          }
          frame "Load Test Procedure" {
            # "#DQMH_CodeNeeded\n1. Configure this Message Case for handling the \"Load Test Procedure\" message.\n2. Delete or edit this label when done."
            # "Loads a test name into memory."
            n168 = Variant To Data(error in=w310, type=T12 {"Test Procedure File Name"=""} ("Load Test Procedure Argument"), Variant=w308) -> (data=w306:T12, error out=w309:errorcluster)
            n169 = Unbundle By Name(w306) -> ("Test Procedure File Name"=w303:string)
            n170 = Bundle By Name(cluster=w305, "Test Procedure File Name"=w303) -> (w304:T5)
          }
          frame "Begin Test Execution" {
            n171 = Variant To Data(error in=w320, type=T13 {"Test Procedure"=""} ("Begin Test Execution Argument"), Variant=w319) -> (data=w317:T13, error out=w312:errorcluster)
            n172 = Unbundle By Name(w317) -> ("Test Procedure"=w314:string)
            n173 = Bundle By Name(cluster=w316, "Test Procedure File Name"=w314) -> (w315:T5)
            n174 = call "Process Test Procedure Metadata.vi"("error in"=w312) -> ("error out"=w311:errorcluster)  [unwired: 10 in]
            n175 = call "Process First Instruction.vi"("error in"=w311) -> ("error out"=w313:errorcluster)  [unwired: 10 in]
          }
          frame "Process Test Procedure Metadata" {
            n176 = Variant To Data(error in=w331, type=T14 {"Boolean"=FALSE} ("Process Test Procedure Metadata Argument"), Variant=w329) -> (data=w327:T14, error out=w330:errorcluster)
            n177 = Unbundle By Name(w324) -> ("Manual Tests Folder"=w326:path, "Test Procedure File Name"=w325:string)
            n178 = Unbundle By Name(w327) -> ()  [unwired: 1 out]
            n179 = call "Process Test Procedure.vi"("Test Procedure File Name"=w325, "Manual Tests Folder"=w326) -> ("TestProcedure"=w322:T2)  [unwired: 9 in]
            "TestProcedure" <- w322
            n180 = Unbundle By Name(w322) -> ("Scope"=w321:string)
            n181 = Bundle By Name(cluster=w324, "TestProcedure"=w322) -> (w323:T5)
            n182 = call "Broadcast Test Scope.vi"("Test Scope"=w321) -> ()  [unwired: 10 in, 1 out]
          }
          frame "Instruction Completed" {
            n183 = Variant To Data(error in=w339, type=T15 {"Boolean"=FALSE} ("Instruction Completed Argument"), Variant=w338) -> (data=w336:T15, error out=w333:errorcluster)
            n184 = Unbundle By Name(w336) -> ()  [unwired: 1 out]
            n185 = in-place {
              n186 = in-place-cluster #4(w335) -> ("TestCaseIndex"=w341:i32)
              n187 = Increment(x=w341) -> (x+1=w340:i32)
              n188 = in-place-cluster #4("TestCaseIndex"=w340) -> (w334:T5)
            }
            n189 = call "Load Next Test Case.vi"("error in"=w333) -> ("error out"=w332:errorcluster)  [unwired: 10 in]
          }
          frame "Process First Instruction" {
            n190 = Variant To Data(error in=w360, type=T16 {"Boolean"=FALSE} ("Process First Instruction Argument"), Variant=w358) -> (data=w356:T16, error out=w359:errorcluster)
            n191 = Unbundle By Name(w356) -> ()  [unwired: 1 out]
            n192 = Unbundle By Name(w349) -> ("Manual Tests Folder"=w355:path, "Test Procedure File Name"=w345:string)
            n193 = call "Process Test Procedure.vi"("Test Procedure File Name"=w345, "Manual Tests Folder"=w355) -> ("TestProcedure"=w347:T2)  [unwired: 9 in]
            n194 = Bundle By Name(cluster=w349, "TestProcedure"=w347) -> (w348:T5)
            n195 = Unbundle By Name(w347) -> ("Section"=w344:string, "Setup Steps"=w354:string[], "Scope"=w343:string)
            n196 = Index Array(array=w354) -> (element=w342:string)  [unwired: 1 in]
            n197 = global write "global.vi" "Test Instruction"(w342) -> ()
            n198 = local write "Scope"(w343) -> ()
            n199 = local write "Instruction"(w342) -> ()
            n200 = call "Refresh Test Procedure Indicator.vi"("Test Procedure"=w345) -> ("error out"=w350:errorcluster)  [unwired: 10 in]
            n201 = call "Refresh Section Indicator.vi"("Section"=w344) -> ("error out"=w351:errorcluster)  [unwired: 10 in]
            n202 = call "Refresh Instruction Indicator.vi"("Instruction"=w342) -> ("error out"=w352:errorcluster)  [unwired: 10 in]
            n203 = call "Broadcast Test Scope.vi"("Test Scope"=w343) -> ("error out"=w353:errorcluster)  [unwired: 10 in]
            n204 = local write "Test Procedure"(w345) -> ()
            n205 = local write "Section"(w344) -> ()
            n206 = Merge Errors(w350, w351, w352, w353) -> (w346:errorcluster)
            n207 = call "Execute Launcher.vi"("error in"=w346) -> ()  [unwired: 10 in, 1 out]
          }
          frame "Load Next Test Case" {
            n208 = Variant To Data(error in=w372, type=T17 {"Boolean"=FALSE} ("Load Next Test Case Argument"), Variant=w370) -> (data=w368:T17, error out=w371:errorcluster)
            n209 = Unbundle By Name(w368) -> ()  [unwired: 1 out]
            n210 = Unbundle By Name(w365) -> ("TestProcedure"=w366:T2, "TestCaseIndex"=w367:i32)
            n211 = Unbundle By Name(w365) -> ("Test Procedure File Name"=w363:string)
            n212 = call "Load Section and Instruction.vi"("TestCaseIndex"=w367, "TestProcedureMetadata"=w366) -> ("Instruction"=w361:string, "Section"=w362:string)  [unwired: 8 in]
            n213 = Empty String/Path?(string/path=w362) -> (empty?=w364:bool)
            n214 = call "Refresh Section Indicator.vi"("Section"=w362) -> ()  [unwired: 10 in, 1 out]
            n215 = case shown="True" w364 {
              tunnel: [_ w373] -> _
              frame False {
              }
              frame True {
                n216 = call "Stop Module.vi"("Wait for Module to Stop? (F)"=TRUE, "Origin"="testCoordinator sent stop") -> ("error out"=w373:errorcluster)  [unwired: 9 in]
              }
            }
            n217 = global write "global.vi" "Test Instruction"(w361) -> ()
            n218 = local write "Test Procedure"(w363) -> ()
            n219 = local write "Section"(w362) -> ()
            n220 = local write "Instruction"(w361) -> ()
            n221 = disable-structure shown="Disabled" {
              disable-tunnel: w362 -> [w376 _]
              frame Disabled {
                n222 = call "Broadcast Actual Test Procedure Section.vi"("Section"=w376) -> ()  [unwired: 10 in, 1 out]
              }
              frame Enabled {
              }
            }
          }
          frame "Execute Launcher" {
            n223 = Variant To Data(error in=w387, type=T18 {"Boolean"=FALSE} ("Execute Launcher Argument"), Variant=w385) -> (data=w383:T18, error out=w378:errorcluster)
            n224 = Unbundle By Name(w383) -> ()  [unwired: 1 out]
            n225 = call "Start Module.vi"("error in"=w378) -> ("error out"=w382:errorcluster, "Wait for Event Sync?"=w381:bool)  [unwired: 6 in, 3 out]
            n226 = call "Synchronize Module Events.vi"("error in"=w382, "Wait for Event Sync?"=w381) -> ("error out"=w380:errorcluster)  [unwired: 9 in]
            n227 = call "Application Mode.vi"("error in"=w380, "Mode"=T23 {"Replay"=enum."None", "Record"=enum."User Events and Benchmarks"}) -> ("error out"=w377:errorcluster)  [unwired: 9 in]
          }
          frame "---Copy This Frame---" {
            # "Duplicate this frame when creating new messages.  Change this comment in the duplicated frame to describe this message."
            n228 = Merge Errors(w390) -> (w389:errorcluster)
          }
          frame "---Exit and Error Handling---" {
            # "Separator - The following cases handle errors and exit messages."
          }
          frame "Simulate MHL Error" {
            # "#DQMH_HowTo The 'Simulate MHL Error' button  illustrates how the MHL handles errors. This event is instructional in nature and can be removed."
            # "Simulate an error occurring at the MHL"
            n229 = call "Module Name--constant.vi"() -> ("Module Name"=w394:string)  [unwired: 11 in]
            n230 = Format Into String(format string="Simulated error originating at Message Handling Loop in %s", w394) -> (resulting string=w395:string)  [unwired: 2 in, 1 out]
            n231 = call <vilib>:"Error Cluster From Error Code.vi"("show call chain? (False)"=TRUE, "error message (\"\")"=w395, "error code (0)"=5001) -> ("error out"=w399:errorcluster)  [unwired: 6 in]
            n232 = Merge Errors(w401, w399) -> (w400:errorcluster)
          }
          frame "Error" {
            # "#DQMH_CodeRecommended - If the module is running in standalone mode (External Launch = FALSE), this code will pop up an error dialog and call the 'Exit' message if an error occurs. Add more fine-grained error management here."
            # "Error - Check the error message data and respond accordingly. This message is sent by the \"Error Handler\" VIs at the end of each loop in this application."
            n233 = property on="Property Node" class="Module Admin"(reference=w404) -> ("Accessors:External Launch"=w403:bool)  [unwired: 1 in, 2 out]
            n234 = Variant To Data(error in=w412, type=errorcluster {"status"=FALSE, "code"=0, "source"=""} ("error constant"), Variant=w406) -> (data=w402:errorcluster, error out=w410:errorcluster)
            n235 = local write "error out"(w402) -> ()
            n236 = call "Error Reported.vi"("Error"=w402) -> ()  [unwired: 10 in, 1 out]
            n237 = case shown="False" w403 {
              tunnel: [w417 _] -> w409
              tunnel: w405 -> [w415 _]
              tunnel: w402 -> [w416 _]
              frame False {
                n238 = disable-structure shown="Default" {
                  disable-tunnel: w416 -> [w418 _]
                  frame condition #0 (active) {
                    # "If the module is running standalone, then pop up an error dialog and call the \"Exit\" message."
                    n239 = call <vilib>:"Simple Error Handler.vi"("error in (no error)"=w418) -> ()  [unwired: 4 in, 5 out]
                  }
                  frame condition #1 {
                    # "To prevent the Simple Error Handler VI from being loaded (e.g. when deploying to a Real-Time target), add the Conditional Disable Symbol \"DQMH_Disable_SEH\" to your project and set it to TRUE."
                  }
                }
                n240 = call-poly <vilib>:"Delacor_lib_QMH_Enqueue Message (poly).vi"("Priority Message? (F)"=TRUE, "Message"="Exit", "Message Queue in"=w415) -> ("error out"=w417:errorcluster)  [unwired: 7 in, 1 out]
              }
              frame True {
                # "If the module was launched externally, calling the Error Reported broadcast VI is the only action performed by the \"Error\" message. The module's caller can then process the error appropriately."
              }
            }
            n241 = Merge Errors(w410, w409) -> (w408:errorcluster)
          }
          frame "Exit" {
            w427 = 91  # 91: not all Exit messages will have an argument
            w429 = TRUE  # Stop the VI
            # "Release the message queue reference"
            # "#DQMH_CodeNeeded - Add any required cleanup code here."
            # "Exit - Exit the application."
            n242 = Variant To Data(error in=w437, type=T10 {"Origin"="", "Exit via Stop Module Req?"=FALSE, "Wait for Module to stop?"=FALSE} ("Stop Argument"), Variant=w428) -> (data=w425:T10, error out=w434:errorcluster)
            n243 = local read "Array"() -> (w420:T1[])
            n244 = call <vilib>:"Clear Errors.vi"("error in (no error)"=w434, "specific error code to clear (0: all)"=w427) -> ("error out"=w436:errorcluster)  [unwired: 4 in, 1 out]
            n245 = control-ref of="This VI"() -> (w424:refnum<vi>)
            n246 = call-dynamic "Delacor_lib_QMH_Release Message Queue.vi"("error in"=w436, "Message Queue"=w431) -> ("error out"=w435:errorcluster)  [unwired: 9 in]
            n247 = call "Handle Exit.vi"("Stop Argument"=w425, "Admin in"=w423, "VI reference"=w424) -> ("error out"=w433:errorcluster)  [unwired: 7 in, 1 out]
            n248 = call "Stop Module.vi"("Wait for Module to Stop? (F)"=TRUE) -> ("error out"=w422:errorcluster)  [unwired: 10 in]
            n249 = call "StoreTestEventsOnRunIDFolder.vi"("Events array"=w420) -> ("error out"=w419:errorcluster)  [unwired: 10 in]
            n250 = Merge Errors(w435, w433, w422, w419) -> (w432:errorcluster)
            n251 = call "Error Reported.vi"("Error"=w432) -> ()  [unwired: 10 in, 1 out]
          }
          frame Default {
            # "'Default' case only runs if there is a message that isn't defined in any of the other cases.  Output a programming error."
            n252 = call "Module Name--constant.vi"() -> ("Module Name"=w442:string)  [unwired: 11 in]
            n253 = Format Into String(format string="The invalid message string \"%s\" was received in the Message Handling Loop for module \"%s\".", w443, w442) -> (resulting string=w438:string)  [unwired: 2 in, 1 out]
            n254 = call <vilib>:"Error Cluster From Error Code.vi"("show call chain? (False)"=TRUE, "error message (\"\")"=w438, "error code (0)"=1) -> ("error out"=w445:errorcluster)  [unwired: 6 in]
            n255 = Merge Errors(w446, w445) -> (w447:errorcluster)
          }
        }
        n256 = call-dynamic "Delacor_lib_QMH_Error Handler - Message Handling Loop.vi"("error in"=w201, "Message Queue in"=w200) -> ("dup error in"=w202:errorcluster)  [unwired: 8 in, 1 out]
      }
    }
    frame Error {
      # "Synchronize Caller Events.vi will inform Start Module.vi that the module has launched and will let the code calling Start Module.vi register for broadcasts and would permit the caller receive the broadcast that an error occurred at launch time."
      n257 = call-dynamic "Delacor_lib_QMH_Release Message Queue.vi"("error in"=w455, "Message Queue"=w448) -> ("error out"=w454:errorcluster)  [unwired: 9 in]
      n258 = call "Synchronize Caller Events.vi"("Singleton Module Admin in"=w449) -> ("error out"=w456:errorcluster)  [unwired: 9 in, 1 out]
      n259 = call "Module Name--constant.vi"() -> ("Module Name"=w452:string)  [unwired: 11 in]
      n260 = Format Into String(format string="An error occurred during initialization. %s is no longer running.", w452) -> (resulting string=w450:string)  [unwired: 2 in, 1 out]
      n261 = Merge Errors(w454, w456) -> (w457:errorcluster)
      n262 = call "Error Reported.vi"("Additional Information"=w450, "Error"=w457) -> ()  [unwired: 9 in, 1 out]
    }
  }
  n263 = Merge Errors(w18, w20) -> (w17:errorcluster)
  n264 = call "Close Module.vi"("error in"=w17, "Module Admin in"=w12) -> ("error out"=w19:errorcluster, "External Launch"=w5:bool, "Module Admin out"=w6:refnum<class "Delacor_lib_QMH_Module Admin.lvclass">)  [unwired: 7 in]
  n265 = Unregister For Events(event registration refnum=w11, error in=w19) -> (error out=w16:errorcluster)
  "error out" <- w16
  n266 = case "External Launch?" shown="True" w5 {
    tunnel: w16 -> [_ w458]
    frame False {
    }
    frame True {
      n267 = case shown="No Error" w458 {
        frame No Error {
          n268 = invoke on="Invoke Node" class="VI" method="FP.Close"() -> ()  [unwired: 3 in, 3 out]
        }
        frame Error {
          n269 = disable-structure shown="Default" {
            frame condition #0 (active) {
              n270 = invoke class="VI" method="FP.Open"("Activate"=TRUE ("Activate?")) -> ()  [unwired: 4 in, 5 out]
            }
            frame condition #1 {
              # "Don't show panel on error if running inside a built EXE."
            }
          }
        }
      }
    }
  }
  n271 = local write "Module Admin"(w6) -> ()
  "Test Procedure" <- w1
  "Section" <- w1
  "Instruction" <- w1
  "Scope" <- w1
